vi "Server Single Connection.vi"() -> ()   [LabVIEW 2026]
doc: "This WebSockets API example VI acts as a server for an incoming websockets connection. Receives/sends string data to the connected client.\nWebSockets 2.0.2.41\nSam Sharp - MediaMongrels Ltd\nCopyright (c) 2023, MediaMongrels Ltd"
uses:
  <vilib>/MediaMongrels Ltd/WebSockets/WebSockets/WebSocket/WebSocket.lvclass/WebSocket.ctl
  <vilib>/MediaMongrels Ltd/WebSockets/WebSockets/WebSocket Server/WebSocket Server.lvclass/WebSocket Server.ctl
  <vilib>/MediaMongrels Ltd/WebSockets/WebSockets/WebSocket/Read Return Headers.vi
  <vilib>/MediaMongrels Ltd/WebSockets/WebSockets/WebSocket Server/Read Request URI.vi
  <vilib>/MediaMongrels Ltd/WebSockets/WebSockets/WebSocket Server/WebSocket Server.lvclass
  <vilib>/MediaMongrels Ltd/WebSockets/Sockets/VISA TCP Listener/VISA TCP Listener.lvclass
panel:
  out "Request URI":string
  out "HTTP Headers":variant
  in  "Stop":bool
  out "Received Data":string
  in  "Send":bool
  in  "Data":string
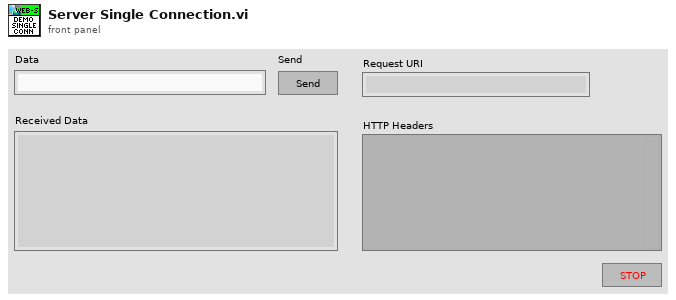
[diagram p1: front panel]
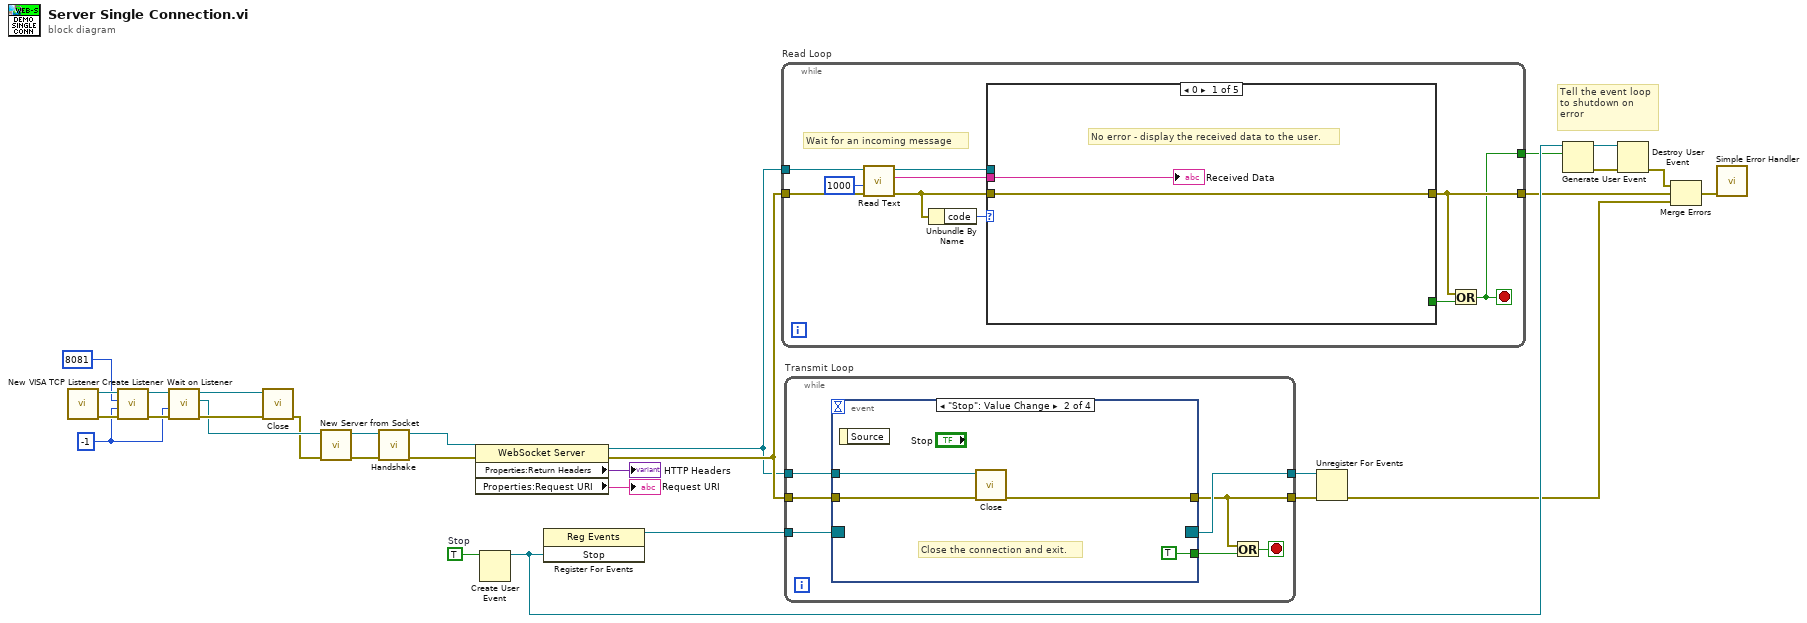
[diagram p0: block diagram]
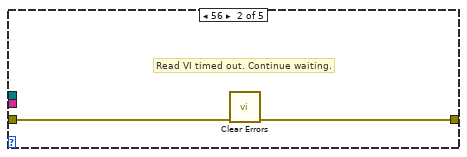
[diagram p2: hidden frame]
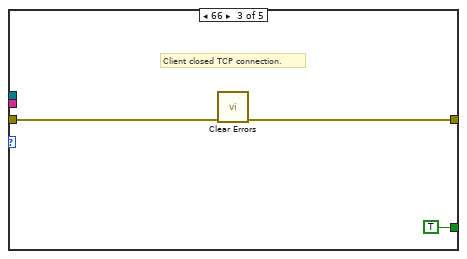
[diagram p3: hidden frame]
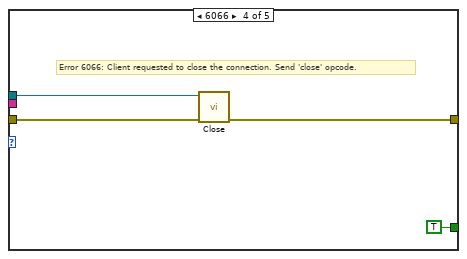
[diagram p4: hidden frame]
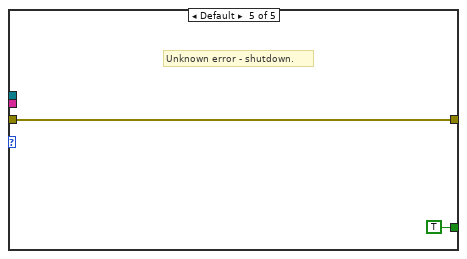
[diagram p5: hidden frame]
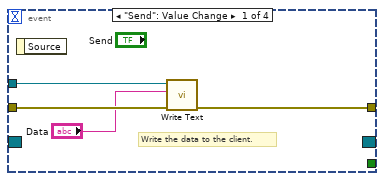
[diagram p6: hidden frame]
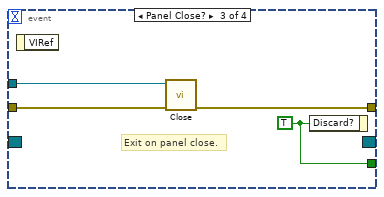
[diagram p7: hidden frame]
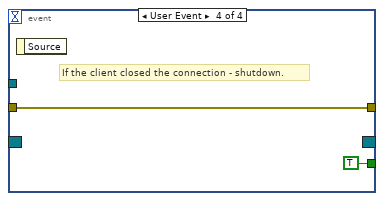
[diagram p8: hidden frame]
diagram:
  w20 = TRUE  # Stop
  w23 = -1 ("timeout ms (25000)")
  # "Tell the event loop to shutdown on error"
  n1 = call <vilib>:"New VISA TCP Listener.vi"() -> ("error out"=w29:errorcluster, "VISA TCP Listener out"=w30:refnum<class "VISA TCP Listener.lvclass">)  [unwired: 10 in]
  n2 = call-dynamic "Create Listener.vi"("error in (no error)"=w29, "timeout ms (5000)"=w23, "Port"=u16 8081 ("port"), "VISA TCP Listener in"=w30) -> ("error out"=w27:errorcluster, "VISA TCP Listener out"=w25:refnum<class "VISA TCP Listener.lvclass">)  [unwired: 6 in]
  n3 = call-dynamic "Wait on Listener.vi"("error in (no error)"=w27, "timeout ms (5000)"=w23, "VISA TCP Listener in"=w25) -> ("error out"=w28:errorcluster, "Socket out"=w22:refnum<class "Socket.lvclass">, "VISA TCP Listener out"=w26:refnum<class "VISA TCP Listener.lvclass">)  [unwired: 6 in]
  n4 = call-dynamic "Close.vi"("error in (no error)"=w28, "VISA TCP Listener in"=w26) -> ("error out"=w7:errorcluster)  [unwired: 9 in]
  n5 = call <vilib>:"New Server from Socket.vi"("error in (no error)"=w7, "Socket"=w22) -> ("error out"=w2:errorcluster, "WebSocket Server out"=w4:refnum<class "WebSocket Server.lvclass">)  [unwired: 8 in]
  n6 = call-dynamic "Handshake.vi"("error in (no error)"=w2, "WebSocket Connection in"=w4) -> ("error out"=w1:errorcluster, "WebSocket Connection out"=w3:refnum<class "WebSocket Server.lvclass">)  [unwired: 8 in]
  n7 = property class="WebSocket Server"(reference=w3, error in=w1) -> (reference out=w8:refnum<class "WebSocket Server.lvclass">, error out=w9:errorcluster, "Properties:Return Headers"=→"HTTP Headers":variant, "Properties:Request URI"=→"Request URI":string)
  n8 = Create User Event(user event datatype=w20) -> (user event=w18:refnum<user-event>)  [unwired: 1 in, 1 out]
  n9 = register-events(w18) -> (reference out=w21:refnum<event-registration>)  [unwired: 2 in, 1 out]
  n10 = while "Read Loop" {
    tunnel: w8 -> [w40]
    tunnel: [w31] -> w17
    tunnel: [w33] -> w11
    tunnel: w9 -> [w34]
    stop <- w31 stop-if-true
    # "Wait for an incoming message"
    n11 = call-dynamic "Read Text.vi"("error in (no error)"=w34, "timeout ms (5000)"=1000 ("timeout ms (25000)"), "WebSocket in"=w40) -> ("error out"=w35:errorcluster, "Data"=w37:string, "WebSocket out"=w36:refnum<class "WebSocket Server.lvclass">)  [unwired: 6 in]
    n12 = Unbundle By Name(w35) -> ("code"=w38:i32)
    n13 = case shown="0" w38 {
      tunnel: w37 -> [w41 _ _ _ _]
      tunnel: [_ _ TRUE TRUE TRUE] -> w32
      tunnel: w36 -> [_ _ _ w51 _]
      tunnel: w35 -> [w42 w44 w46 w49 w52]
      tunnel: [w42 w43 w45 w48 w52] -> w33
      frame 0 {
        # "No error - display the received data to the user."
        "Received Data" <- w41
      }
      frame 56 {
        # "Read VI timed out. Continue waiting."
        n14 = call <vilib>:"Clear Errors.vi"("error in (no error)"=w44) -> ("error out"=w43:errorcluster)  [unwired: 5 in, 1 out]
      }
      frame 66 {
        # "Client closed TCP connection."
        n15 = call <vilib>:"Clear Errors.vi"("error in (no error)"=w46) -> ("error out"=w45:errorcluster)  [unwired: 5 in, 1 out]
      }
      frame 6066 {
        # "Error 6066: Client requested to close the connection. Send 'close' opcode."
        n16 = call-dynamic "Close.vi"("error in (no error)"=w49, "WebSocket in"=w51) -> ("error out"=w48:errorcluster)  [unwired: 9 in]
      }
      frame Default {
        # "Unknown error - shutdown."
      }
    }
    n17 = Or(x=w33, y=w32) -> (x .or. y?=w31:bool)
  }
  n18 = while "Transmit Loop" {
    tunnel: w8 -> [w60]
    tunnel: w21 -> [w59]
    tunnel: [w58] -> w19
    tunnel: [w54] -> w12
    tunnel: w9 -> [w57]
    stop <- w55 stop-if-true
    n19 = event shown="[1] \"Stop\": Value Change" {
      selector: w59 -> [_ _ _ _]
      dyn-events: [_ _ _ _] -> w58
      timeout: _ -> [_ _ _ _]
      tunnel: w60 -> [w64 w67 w72 _]
      tunnel: [_ TRUE w71 TRUE] -> w56
      tunnel: [w62 w66 w70 w73] -> w54
      tunnel: w57 -> [w63 w65 w69 w73]
      event "Send": Value Change {
        # "Write the data to the client."
        n20 = event-data() -> ()  [unwired: 1 in, 1 out]
        n21 = call-dynamic "Write Text.vi"("error in (no error)"=w63, "String Data"="Data", "WebSocket in"=w64) -> ("error out"=w62:errorcluster)  [unwired: 7 in, 1 out]
      }
      event "Stop": Value Change {
        # "Close the connection and exit."
        n22 = event-data() -> ()  [unwired: 1 in, 1 out]
        n23 = call-dynamic "Close.vi"("error in (no error)"=w65, "WebSocket in"=w67) -> ("error out"=w66:errorcluster)  [unwired: 9 in]
      }
      event Panel Close? {
        w71 = TRUE ("Discard?")
        # "Exit on panel close."
        n24 = event-data() -> ()  [unwired: 1 in, 1 out]
        n25 = call-dynamic "Close.vi"("error in (no error)"=w69, "WebSocket in"=w72) -> ("error out"=w70:errorcluster)  [unwired: 9 in]
        n26 = event-data("Discard?"=w71) -> ()  [unwired: 1 in, 1 out]
      }
      event User Event {
        # "If the client closed the connection - shutdown."
        n27 = event-data() -> ()  [unwired: 1 in, 1 out]
      }
    }
    n28 = Or(x=w54, y=w56) -> (x .or. y?=w55:bool)
  }
  n29 = Unregister For Events(event registration refnum=w19, error in=w12) -> (error out=w10:errorcluster)
  n30 = Generate User Event(user event=w18, event data cluster=w17) -> (user event out=w16:refnum<user-event>, error out=w15:errorcluster)  [unwired: 2 in]
  n31 = Destroy User Event(user event=w16, error in=w15) -> (error out=w14:errorcluster)
  n32 = Merge Errors(w14, w11, w10) -> (w13:errorcluster)
  n33 = call <vilib>:"Simple Error Handler.vi"("error in (no error)"=w13) -> ()  [unwired: 4 in, 5 out]
